vi "query Input Signal Overload.vi"(8 "error in (no error)":errorcluster, 11 "Keysight 9020A in":refnum<class "Keysight 9020A.lvclass">) -> (0 "error out":errorcluster, 2 "Input Overload?":bool, 3 "Keysight 9020A out":refnum<class "Keysight 9020A.lvclass">)   [LabVIEW 2023, in "Spectrum Analyzer.lvlib" / "Keysight 9020A.lvclass"]
uses:
  Keysight 9020A.lvclass
  Keysight 9020A.lvclass/Keysight 9020A.ctl
  Spectrum Analyzer.lvlib
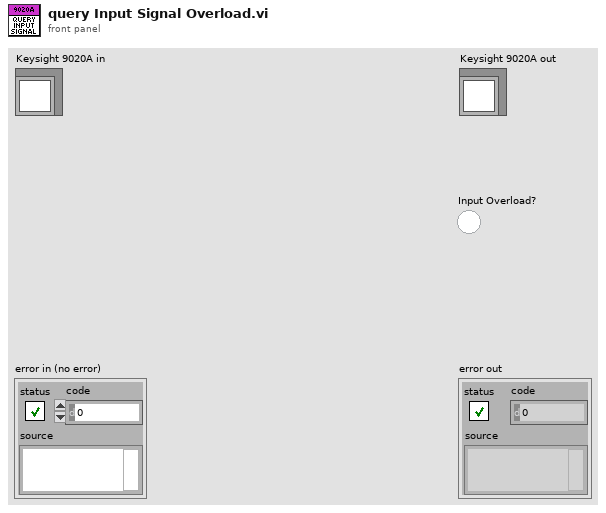
[diagram p1: front panel]
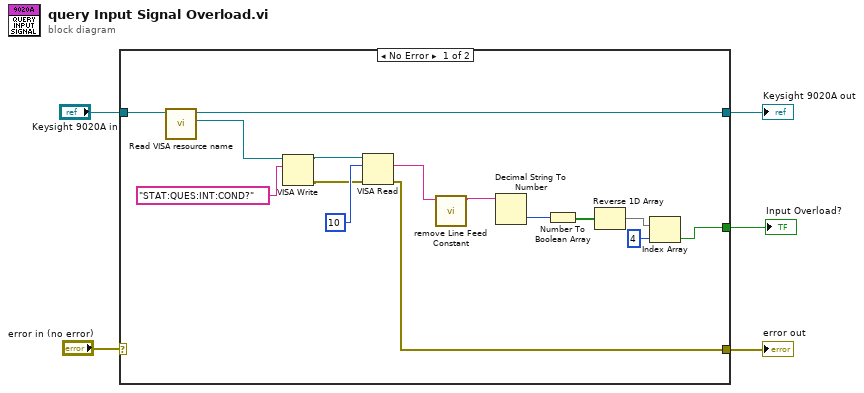
[diagram p0: block diagram]
diagram:
  n1 = case shown="No Error" "error in (no error)" {
    selector: "error in (no error)" -> [_ w21]
    tunnel: "Keysight 9020A in" -> [w18 w22]
    tunnel: [w20 w22] -> w4
    tunnel: [w7 w21] -> w3
    tunnel: [w6 _] -> w1
    frame No Error {
      n2 = call "Read VISA resource name.vi"("Keysight 9020A in"=w18) -> ("VISA resource name"=w19:refnum<visa-resource-name>, "Keysight 9020A out"=w20:refnum<class "Keysight 9020A.lvclass">)  [unwired: 8 in, 1 out]
      n3 = VISA Write(VISA resource name=w19, write buffer="STAT:QUES:INT:COND?") -> (VISA resource name out=w11:refnum<visa-resource-name>, error out=w10:errorcluster)  [unwired: 1 in, 1 out]
      n4 = VISA Read(VISA resource name=w11, byte count=u32 10, error in (no error)=w10) -> (read buffer=w9:string, error out=w7:errorcluster)  [unwired: 2 out]
      n5 = call "remove Line Feed Constant.vi"("Input String"=w9) -> ("Line Feed Removed String"=w8:string)  [unwired: 10 in]
      n6 = Decimal String To Number(string=w8) -> (number=w14:i32)  [unwired: 2 in, 1 out]
      n7 = Number To Boolean Array(number=w14) -> (Boolean array=w15:bool[])
      n8 = Reverse 1D Array(array=w15) -> (reversed array=w13:bool[])
      n9 = Index Array(array=w13, index=4) -> (element=w6:bool)
    }
    frame Error {
    }
  }
  "error out" <- w3
  "Keysight 9020A out" <- w4
  "Input Overload?" <- w1
